vi "Sample Test.vi"(4 "Execution time (s)":dbl=-1.0, 8 "error in (no error)":errorcluster) -> (0 "error out":errorcluster)   [LabVIEW 2020]
uses:
  classes/Assert/Assert False.vi
  classes/Test/Test.lvclass
  classes/Assert/Assert.lvclass
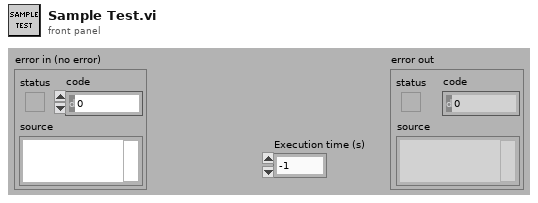
[diagram p1: front panel]
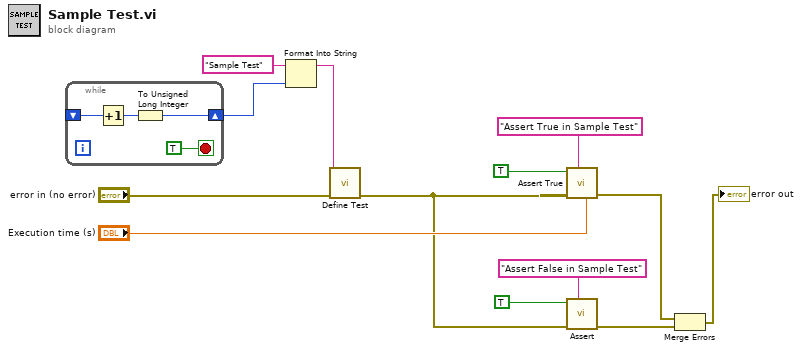
[diagram p0: block diagram]
diagram:
  n1 = while {
    shift-right: [w15] -> w10
    shift-left: _ -> [w17]
    stop <- TRUE stop-if-true
    n2 = Increment(x=w17) -> (x+1=w16:u32)
    n3 = To Unsigned Long Integer(number=w16) -> (unsigned 32bit integer=w15:u32)
  }
  n4 = Format Into String(initial string="Sample Test" ("Label (VI Title)"), w10) -> (resulting string=w9:string)  [unwired: 2 in, 1 out]
  n5 = call "Define Test.vi"("error in (no error)"="error in (no error)", "Label (VI Title)"=w9) -> ("error out"=w4:errorcluster)  [unwired: 8 in, 1 out]
  n6 = call "Assert True.vi"("Execution time (s)"="Execution time (s)", "Label"="Assert True in Sample Test", "error in (no error)"=w4, "True?"=TRUE) -> ("error out"=w7:errorcluster)  [unwired: 6 in, 1 out]
  n7 = call-poly "Assert.vi"("Label"="Assert False in Sample Test", "error in (no error)"=w4, "False?"=TRUE ("True?")) -> ("error out"=w2:errorcluster)  [unwired: 7 in, 1 out]
  n8 = Merge Errors(w7, w2) -> (→"error out":errorcluster)
